vi "Wire Selected_Index To Case Selector.vi"(8 "error in (no error)":errorcluster, 9 "CaseStructure in":refnum<vi>, 10 "SubVI in":refnum<vi>, 11 "Unbundler in":refnum<vi>) -> (0 "error out":errorcluster, 1 "Case Structure out":refnum<vi>, 2 "SubVI out":refnum<vi>, 3 "Unbundler out":refnum<vi>)   [LabVIEW 2019, in "gRPC Template Creation Utility.lvlib"]
uses:
  gRPC Template Creation Utility.lvlib
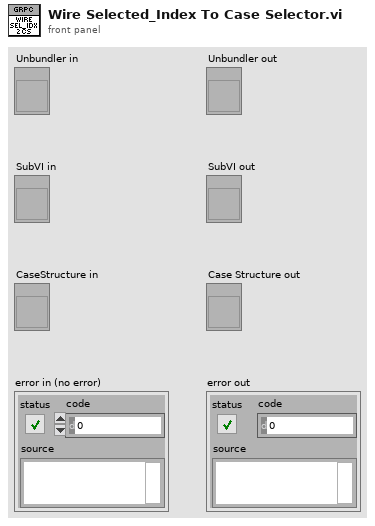
[diagram p1: front panel]
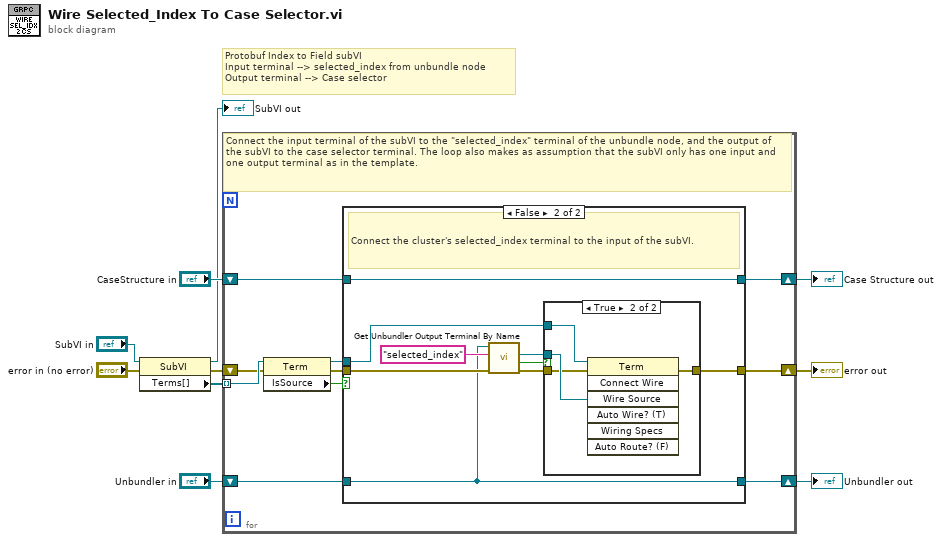
[diagram p0: block diagram]
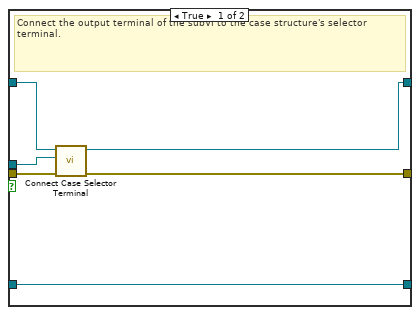
[diagram p2: hidden frame]
diagram:
  # "Protobuf Index to Field subVI\nInput terminal --> selected_index from unbundle node\nOutput terminal --> Case selector"
  n1 = property class="SubVI"(reference="SubVI in", error in="error in (no error)") -> (reference out=→"SubVI out":refnum<vi>, error out=w10:errorcluster, "Terms[]"=w6:refnum<vi>[])
  n2 = for {
    tunnel: w6 -> [w16] mode=indexing
    shift-right: [w14] -> w9
    shift-left: w10 -> [w13]
    shift-right: [w11] -> w1
    shift-left: "Unbundler in" -> [w19]
    shift-right: [w12] -> w2
    shift-left: "CaseStructure in" -> [w15]
    # "Connect the input terminal of the subVI to the \"selected_index\" terminal of the unbundle node, and the output of the subVI to the case selector terminal. The loop also makes as assumption that the subVI only has one input and one output terminal as in the template."
    n3 = property class="Term"(reference=w16, error in=w13) -> (reference out=w17:refnum<vi>, error out=w18:errorcluster, "IsSource"=w20:bool)
    n4 = case shown="False" w20 {
      tunnel: w19 -> [w21 w27]
      tunnel: w18 -> [w24 w35]
      tunnel: w17 -> [w25 w34]
      tunnel: w15 -> [w26 w28]
      tunnel: [w23 w30] -> w14
      tunnel: [w22 w28] -> w12
      tunnel: [w21 w27] -> w11
      frame True {
        # "Connect the output terminal of the subVI to the case structure's selector terminal."
        n5 = call "Connect Case Selector Terminal.vi"("error in (no error)"=w24, "Wire Source"=w25, "Case Structure in"=w26) -> ("error IO"=w23:errorcluster, "Case Structure out"=w22:refnum<vi>)  [unwired: 7 in]
      }
      frame False {
        # "Connect the cluster's selected_index terminal to the input of the subVI."
        n6 = call "Get Unbundler Output Terminal By Name.vi"("error in (no error)"=w35, "Terminal name"="selected_index" ("String"), "Unbundler in"=w27) -> ("error out"=w31:errorcluster, "Found?"=w32:bool, "Terminal Refnum"=w33:refnum<vi>)  [unwired: 5 in, 1 out]
        n7 = case shown="True" w32 {
          tunnel: w34 -> [_ w40]
          tunnel: w33 -> [_ w39]
          tunnel: w31 -> [w36 w38]
          tunnel: [w36 w37] -> w30
          frame False {
          }
          frame True {
            n8 = invoke class="Term" method="Connect Wire"(reference=w40, error in=w38, "Wire Source"=w39) -> (error out=w37:errorcluster)  [unwired: 4 in, 6 out]
          }
        }
      }
    }
  }
  "error out" <- w9
  "Case Structure out" <- w2
  "Unbundler out" <- w1
